vi "FGV_new.vi"(9 "目标时间":dbl=inf, 10 "动作":enum16{"开始计时", "暂停", "继续"}(ring)) -> (1 "是否超时":bool, 2 "进度":dbl, 3 "计时时间":dbl)   [LabVIEW 2026, in "UI-无创.lvlib"]
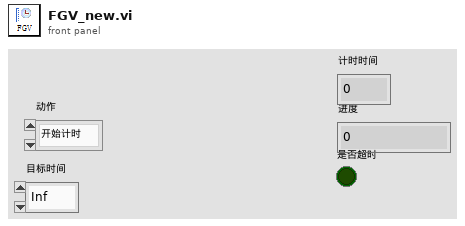
[diagram p1: front panel]
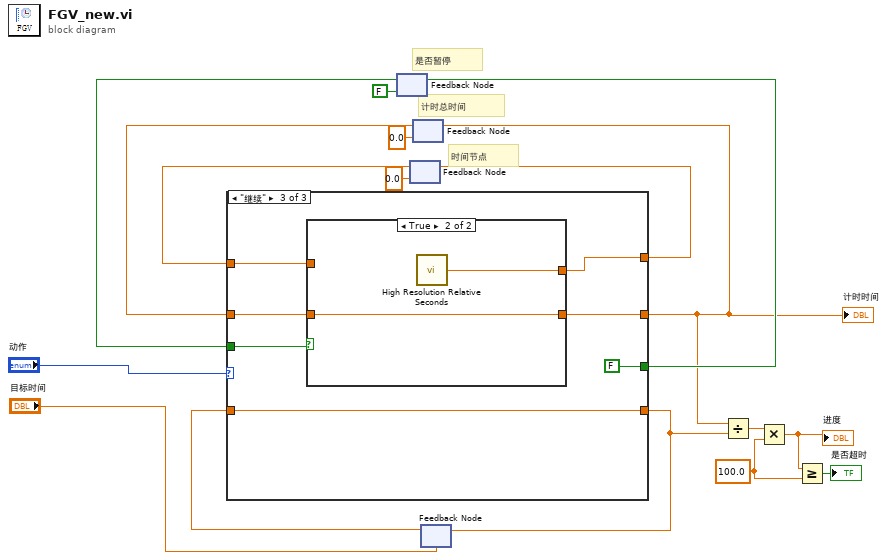
[diagram p0: block diagram]
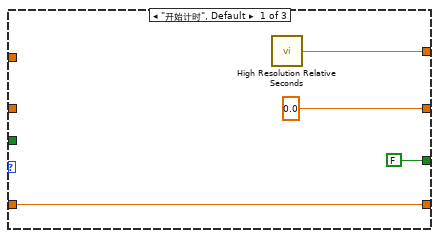
[diagram p2: hidden frame]
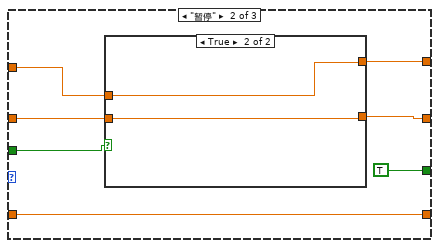
[diagram p3: hidden frame]
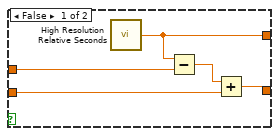
[diagram p4: hidden frame]
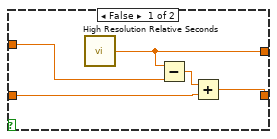
[diagram p5: hidden frame]
diagram:
  w1 = 100.0 ("y")
  # "是否暂停"
  # "时间节点"
  # "计时总时间"
  n1 = feedback #1(FALSE) -> (w12:bool)
  n2 = feedback #2(0.0 ("relative seconds")) -> (w15:dbl)
  n3 = feedback #3(0.0) -> (w14:dbl)
  n4 = feedback #4("目标时间") -> (w8:dbl)
  n5 = case shown="\"继续\"" "动作" {
    tunnel: [w21 w27 w40] -> w16
    tunnel: w15 -> [_ w28 w38]
    tunnel: w8 -> [w18 w22 w36]
    tunnel: [0.0 w25 w37] -> w10
    tunnel: w14 -> [_ w26 w39]
    tunnel: [FALSE TRUE FALSE] -> w13
    tunnel: w12 -> [_ w24 w41]
    tunnel: [w18 w22 w36] -> w7
    frame "开始计时", Default {
      n6 = call <vilib>:"High Resolution Relative Seconds.vi"() -> ("relative seconds"=w21:dbl)
    }
    frame "暂停" {
      n7 = case shown="True" w24 {
        tunnel: w28 -> [w33 w35]
        tunnel: [w32 w35] -> w27
        tunnel: w26 -> [w31 w34]
        tunnel: [w29 w34] -> w25
        frame False {
          n8 = call <vilib>:"High Resolution Relative Seconds.vi"() -> ("relative seconds"=w32:dbl)
          n9 = Subtract(x=w32, y=w33) -> (x-y=w30:dbl)
          n10 = Add(x=w30, y=w31) -> (x+y=w29:dbl)
        }
        frame True {
        }
      }
    }
    frame "继续" {
      n11 = case shown="True" w41 {
        tunnel: [w47 w49] -> w40
        tunnel: [w43 w48] -> w37
        tunnel: w39 -> [w44 w48]
        tunnel: w38 -> [w46 _]
        frame False {
          n12 = call <vilib>:"High Resolution Relative Seconds.vi"() -> ("relative seconds"=w47:dbl)
          n13 = Subtract(x=w47, y=w46) -> (x-y=w45:dbl)
          n14 = Add(x=w45, y=w44) -> (x+y=w43:dbl)
        }
        frame True {
          n15 = call <vilib>:"High Resolution Relative Seconds.vi"() -> ("relative seconds"=w49:dbl)
        }
      }
    }
  }
  "计时时间" <- w10
  n16 = feedback-in #1(w13) -> ()
  n17 = feedback-in #2(w16) -> ()
  n18 = feedback-in #3(w10) -> ()
  n19 = feedback-in #4(w7) -> ()
  n20 = Divide(x=w10, y=w7) -> (x/y=w9:dbl)
  n21 = Multiply(x=w9, y=w1) -> (x*y=w2:dbl)
  "进度" <- w2
  n22 = Greater Or Equal?(x=w2, y=w1) -> (x >= y?=→"是否超时":bool)
